vi "test unsupported version id.vi"(8 "error in (no error)":errorcluster) -> (0 "error out":errorcluster, 3 "body":string)   [LabVIEW 2020, in "MCP Server tests.lvlib"]
doc: "An MCP-Protocol-Version header the server does not support is refused before the body is handled: HTTP 400 with the JSON-RPC error -32022. The refusal carries the id of the request - a number stays a number, a string stays a string - instead of null. Sent on a legacy tools/list (id 681 and id \"v68\") and on a modern server/discover whose header and _meta say v999.0.0 (id 682, data.requested v999.0.0). The requests are sent with the LabVIEW HTTP Client directly."
uses:
  MCP Server tests.lvlib
  <vilib>/addons/_JKI Toolkits/Caraya/classes/Test/Test.lvclass
  <vilib>/addons/_JKI Toolkits/Caraya/classes/Assert/Assert.lvclass
panel:
  out "lookup error":errorcluster
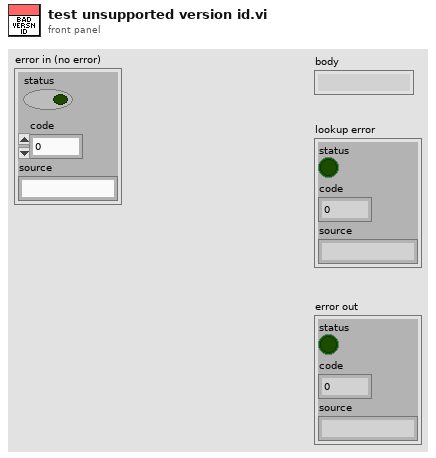
[diagram p1: front panel]
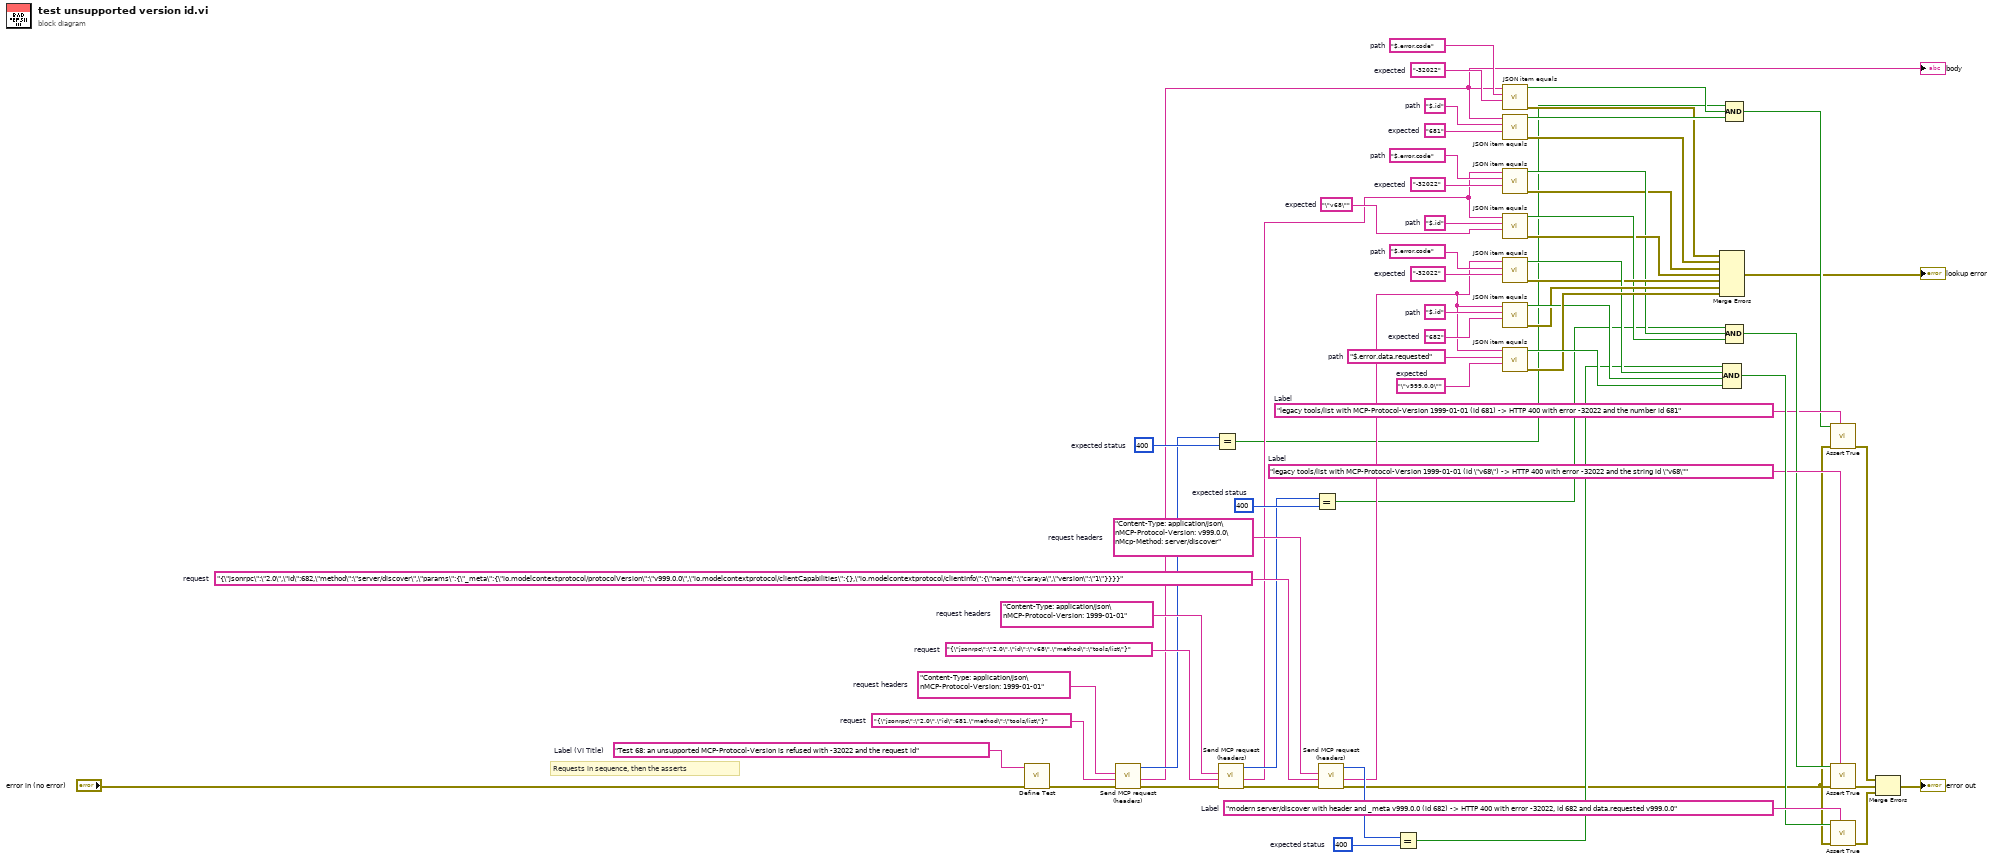
[diagram p0: block diagram]
diagram:
  w61 = "modern server/discover with header and _meta v999.0.0 (id 682) -> HTTP 400 with error -32022, id 682 and data.requested v999.0.0"  # Label
  w58 = "legacy tools/list with MCP-Protocol-Version 1999-01-01 (id \"v68\") -> HTTP 400 with error -32022 and the string id \"v68\""  # Label
  w55 = "legacy tools/list with MCP-Protocol-Version 1999-01-01 (id 681) -> HTTP 400 with error -32022 and the number id 681"  # Label
  w50 = "\"v999.0.0\""  # expected
  w49 = "$.error.data.requested"  # path
  w46 = "682"  # expected
  w45 = "$.id"  # path
  w42 = "-32022"  # expected
  w41 = "$.error.code"  # path
  w39 = 400  # expected status
  w35 = "Content-Type: application/json\nMCP-Protocol-Version: v999.0.0\nMcp-Method: server/discover"  # request headers
  w34 = "{\"jsonrpc\":\"2.0\",\"id\":682,\"method\":\"server/discover\",\"params\":{\"_meta\":{\"io.modelcontextprotocol/protocolVersion\":\"v999.0.0\",\"io.modelcontextprotocol/clientCapabilities\":{},\"io.modelcontextprotocol/clientInfo\":{\"name\":\"caraya\",\"version\":\"1\"}}}}"  # request
  w31 = "\"v68\""  # expected
  w30 = "$.id"  # path
  w27 = "-32022"  # expected
  w26 = "$.error.code"  # path
  w24 = 400  # expected status
  w20 = "Content-Type: application/json\nMCP-Protocol-Version: 1999-01-01"  # request headers
  w19 = "{\"jsonrpc\":\"2.0\",\"id\":\"v68\",\"method\":\"tools/list\"}"  # request
  w16 = "681"  # expected
  w15 = "$.id"  # path
  w12 = "-32022"  # expected
  w11 = "$.error.code"  # path
  w9 = 400  # expected status
  w5 = "Content-Type: application/json\nMCP-Protocol-Version: 1999-01-01"  # request headers
  w4 = "{\"jsonrpc\":\"2.0\",\"id\":681,\"method\":\"tools/list\"}"  # request
  w2 = "Test 68: an unsupported MCP-Protocol-Version is refused with -32022 and the request id"  # Label (VI Title)
  # "Requests in sequence, then the asserts"
  n1 = call <vilib>:"Define Test.vi"("error in (no error)"="error in (no error)", "Label (VI Title)"=w2) -> ("error out"=w3:errorcluster)  [unwired: 8 in, 1 out]
  n2 = call "Send MCP request (headers).vi"("error in (no error)"=w3, "request"=w4, "request headers"=w5) -> ("error out"=w6:errorcluster, "response"=w7:string, "status code"=w8:i32)  [unwired: 5 in, 1 out]
  "body" <- w7
  n3 = Equal?(x=w8, y=w9) -> (x = y?=w10:bool)
  n4 = call "Send MCP request (headers).vi"("error in (no error)"=w6, "request"=w19, "request headers"=w20) -> ("error out"=w21:errorcluster, "response"=w22:string, "status code"=w23:i32)  [unwired: 5 in, 1 out]
  n5 = Equal?(x=w23, y=w24) -> (x = y?=w25:bool)
  n6 = call "Send MCP request (headers).vi"("error in (no error)"=w21, "request"=w34, "request headers"=w35) -> ("error out"=w36:errorcluster, "response"=w37:string, "status code"=w38:i32)  [unwired: 5 in, 1 out]
  n7 = Equal?(x=w38, y=w39) -> (x = y?=w40:bool)
  n8 = call "JSON item equals.vi"("expected"=w12, "path"=w11, "JSON"=w7) -> ("error out"=w13:errorcluster, "equal?"=w14:bool)  [unwired: 6 in, 1 out]
  n9 = call "JSON item equals.vi"("expected"=w16, "path"=w15, "JSON"=w7) -> ("error out"=w17:errorcluster, "equal?"=w18:bool)  [unwired: 6 in, 1 out]
  n10 = call "JSON item equals.vi"("expected"=w27, "path"=w26, "JSON"=w22) -> ("error out"=w28:errorcluster, "equal?"=w29:bool)  [unwired: 6 in, 1 out]
  n11 = call "JSON item equals.vi"("expected"=w31, "path"=w30, "JSON"=w22) -> ("error out"=w32:errorcluster, "equal?"=w33:bool)  [unwired: 6 in, 1 out]
  n12 = call "JSON item equals.vi"("expected"=w42, "path"=w41, "JSON"=w37) -> ("error out"=w43:errorcluster, "equal?"=w44:bool)  [unwired: 6 in, 1 out]
  n13 = call "JSON item equals.vi"("expected"=w46, "path"=w45, "JSON"=w37) -> ("error out"=w47:errorcluster, "equal?"=w48:bool)  [unwired: 6 in, 1 out]
  n14 = call "JSON item equals.vi"("expected"=w50, "path"=w49, "JSON"=w37) -> ("error out"=w51:errorcluster, "equal?"=w52:bool)  [unwired: 6 in, 1 out]
  n15 = Merge Errors(w13, w17, w28, w32, w43, w47, w51) -> (→"lookup error":errorcluster)
  n16 = Compound Arithmetic op=AND(w40, w44, w48, w52) -> (w60:bool)
  n17 = Compound Arithmetic op=AND(w10, w14, w18) -> (w54:bool)
  n18 = Compound Arithmetic op=AND(w25, w29, w33) -> (w57:bool)
  n19 = call <vilib>:"Assert True.vi"("Label"=w55, "error in (no error)"=w36, "True?"=w54) -> ("error out"=w56:errorcluster)  [unwired: 7 in, 1 out]
  n20 = call <vilib>:"Assert True.vi"("Label"=w58, "error in (no error)"=w36, "True?"=w57) -> ("error out"=w59:errorcluster)  [unwired: 7 in, 1 out]
  n21 = call <vilib>:"Assert True.vi"("Label"=w61, "error in (no error)"=w36, "True?"=w60) -> ("error out"=w62:errorcluster)  [unwired: 7 in, 1 out]
  n22 = Merge Errors(w56, w59, w62) -> (→"error out":errorcluster)
